vi "Set Result.vi"(8 "error in (no error)":errorcluster, 9 "dS":dbl, 10 "XY Plot":refnum<vi>, 11 "4way Lap in":refnum<class "4way Lap.lvclass">) -> (0 "error out":errorcluster, 3 "4way Lap out":refnum<class "4way Lap.lvclass">)   [LabVIEW 2025, in "Flow Grind.lvlib" / "4way Lap.lvclass"]
uses:
  4way Lap.lvclass
  FG configuration/FlowGrind configuration.lvclass
  4way Lap.lvclass/4way Lap.ctl
  FG configuration/FlowGrind configuration.lvclass/FlowGrind configuration.ctl
  FG configuration/Read FlowGrind.vi
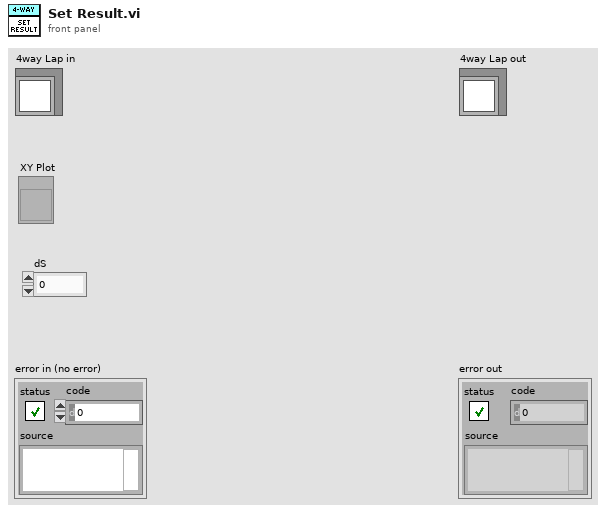
[diagram p1: front panel]
types:
  T1 = cluster{"Name":string, "Color":u32, "Style":u8, "Point Style":u8, "Name Visible":bool, "Allow Drag":bool, "Annotation Mode":u32, "Plot":i32, "Index":i32, "Position":cluster{"X":dbl, "Y":dbl}, "X Scale":u32, "Y Scale":u32, "Show Arrow":bool, "Lock Name":bool, "Plot Area":i32, "Label Offset":cluster{"X":dbl, "Y":dbl}}
  T2 = typedef "Flow Grind.lvlib/FlowGrind configuration.lvclass/FlowGrind Settings.ctl" = cluster{"Build Profile":cluster{"Ramp Start":dbl, "Ramp End":dbl, "Ramp Rate Far":dbl, "Ramp Rate Close":dbl, "Null Lower Limit":dbl, "Null Upper Limit":dbl, "Test Mode":string}[][], "Scale Factor":cluster{"X":dbl, "Y":dbl}, "Lap Condition":dbl, "Supply Pressure":dbl, "Simulated?":bool}
  T3 = typedef "LVAnnotationListTypeDef.ctl" = cluster{"Name":string, "Color":u32, "Style":u8, "Point Style":u8, "Name Visible":bool, "Allow Drag":bool, "Annotation Mode":u32, "Plot":i32, "Index":i32, "Position":cluster{"X":dbl, "Y":dbl}, "X Scale":u32, "Y Scale":u32, "Show Arrow":bool, "Lock Name":bool, "Plot Area":i32, "Label Offset":cluster{"X":dbl, "Y":dbl}}[]
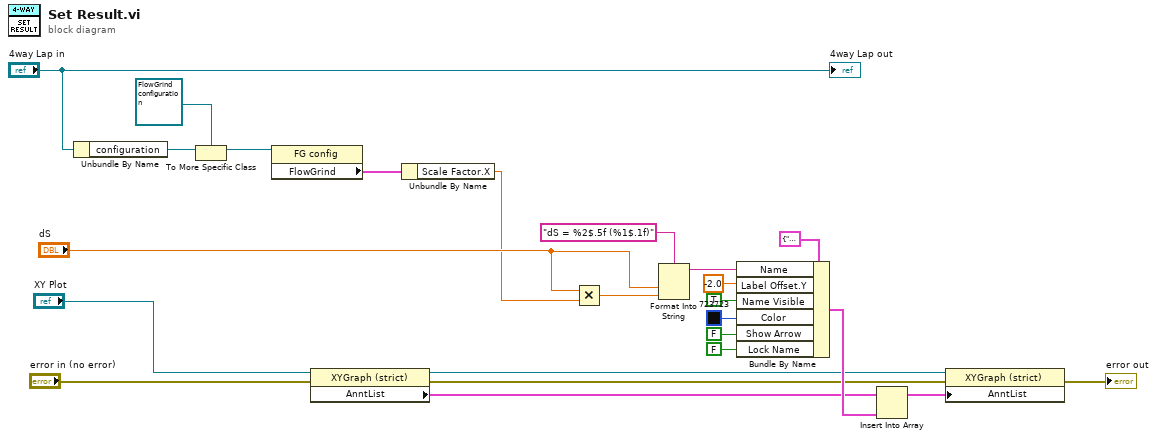
[diagram p0: block diagram]
diagram:
  n1 = Unbundle By Name("4way Lap in") -> ("configuration"=w8:refnum<class "FlowGrind configuration.lvclass">)
  n2 = To More Specific Class(target class=refnum<class "FlowGrind configuration.lvclass"> refnum ("Flow Grind.lvlib:XY Plotter config"), reference=w8) -> (specific class reference=w7:refnum<class "FlowGrind configuration.lvclass">)  [unwired: 1 in, 1 out]
  n3 = property class="FG config"(reference=w7) -> ("FlowGrind"=w6:T2)  [unwired: 1 in, 2 out]
  n4 = property class="XYGraph (strict)"(reference="XY Plot", error in="error in (no error)") -> (reference out=w18:refnum<vi>, error out=w20:errorcluster, "AnntList"=w19:T3)
  n5 = Unbundle By Name(w6) -> ("Scale Factor.X"=w2:dbl)
  n6 = Multiply(x="dS", y=w2) -> (x*y=w1:dbl)
  n7 = Format Into String(format string="dS = %2$.5f (%1$.1f)", "dS", w1) -> (resulting string=w17:string)  [unwired: 2 in, 1 out]
  n8 = Bundle By Name(cluster=T1 {"Name"="", "Color"=0, "Style"=0, "Point Style"=0, "Name Visible"=FALSE, "Allow Drag"=FALSE, "Annotation Mode"=0, "Plot"=0, "Index"=0, "Position"={"X"=0.0, "Y"=0.0}, "X Scale"=0, "Y Scale"=0, "Show Arrow"=FALSE, "Lock Name"=FALSE, "Plot Area"=0, "Label Offset"={"X"=0.0, "Y"=0.0}} ("new element/subarray"), "Name"=w17, "Label Offset.Y"=-2.0, "Name Visible"=TRUE, "Color"=u32 723723, "Show Arrow"=FALSE, "Lock Name"=FALSE) -> (w23:T1)
  n9 = Insert Into Array(array=w19, new element=w23) -> (w21:T3)  [unwired: 1 in]
  n10 = property class="XYGraph (strict)"(reference=w18, error in=w20, "AnntList"=w21) -> (error out=→"error out":errorcluster)  [unwired: 1 out]
  "4way Lap out" <- "4way Lap in"
